vi "DIO-DAQ-Panel.vi"(7 "Set(F)":bool, 8 "error in (no error)":errorcluster, 10 "First Time(F)":bool, 11 "object in":refnum<class>) -> (0 "error out":errorcluster, 2 "Changed?":bool, 3 "object out":refnum<class>)   [LabVIEW 2021, in "DAQmx.lvlib" / "DIO-Configuration.lvclass"]
uses:
  DIO-Configuration.lvclass
  Dependencies/DIO-Channel.lvlibp/Channels/DIO-Channel/DIO-Configuration_class/tdef/Direction.ctl
  C:/Users/averna/Documents/LV Gym DEMO/Factory Pattern/Device Channels/Dependencies/DIO-Channel.lvlibp/Channels/DIO-Channel/DIO-Configuration_class/DIO-Configuration.lvclass
  tdef/Data.ctl
  DAQmx.lvlib
  Dependencies/DIO-Channel.lvlibp/Channels/DIO-Channel/DIO-Configuration_class/DIO-Configuration.lvclass
panel:
  in  "Direction":T1
  in  "Line":string(combo)
  in  "Device":string(combo)
  out "Not Saved?":bool
  in  "Save":bool
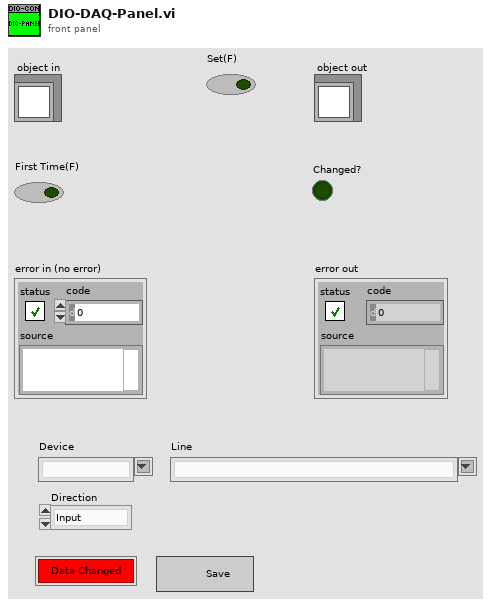
[diagram p1: front panel]
types:
  T1 = typedef "DIO-Channel.lvlibp/DIO-Configuration.lvclass/Direction.ctl" = enum16{"Input", "Output"}
  T2 = typedef "DAQmx.lvlib/DIO-Configuration.lvclass/Data.ctl" = cluster{"DAQ_Line":string}
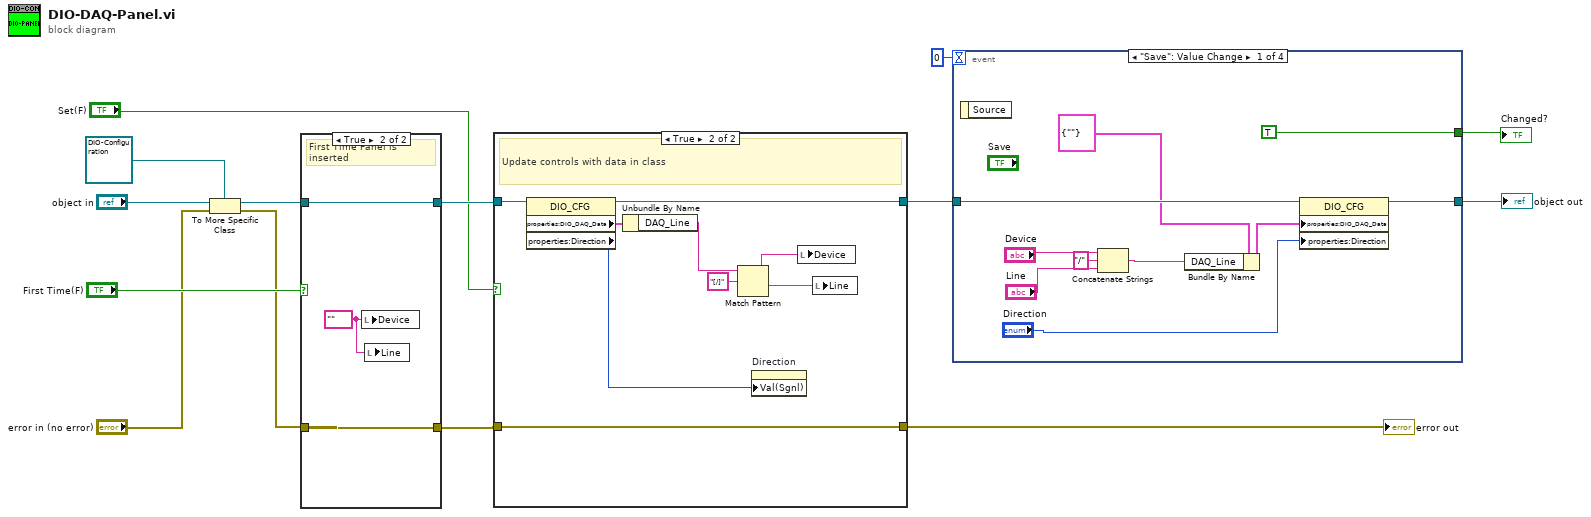
[diagram p0: block diagram]
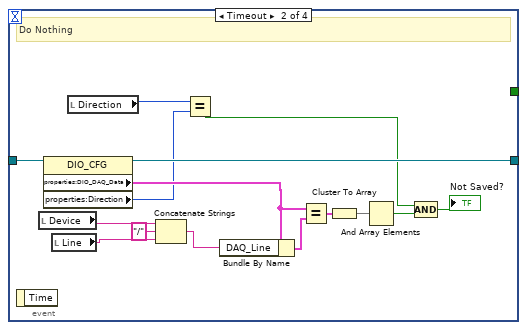
[diagram p3: hidden frame]
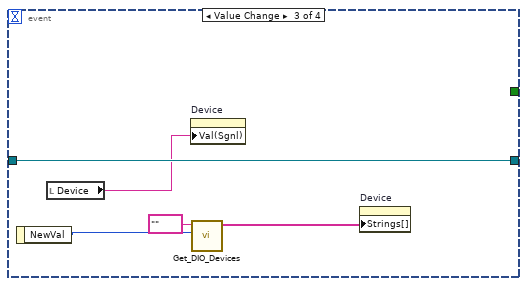
[diagram p4: hidden frame]
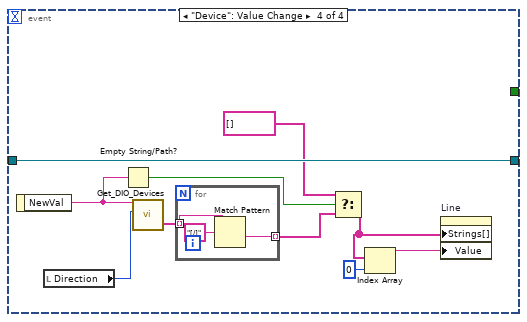
[diagram p5: hidden frame]
diagram:
  n1 = To More Specific Class(target class=refnum<class "DIO-Configuration.lvclass"> refnum ("Template-Channels.lvlib:Template_CFG"), reference="object in", error in="error in (no error)") -> (specific class reference=w8:refnum<class "DIO-Configuration.lvclass">, error out=w6:errorcluster)
  n2 = case shown="True" "First Time(F)" {
    tunnel: [w16 w19] -> w12
    tunnel: w8 -> [w16 w19]
    tunnel: [w15 w18] -> w11
    tunnel: w6 -> [w15 w18]
    frame False {
    }
    frame True {
      w17 = "" ("Device")
      # "First Time Panel is inserted"
      n3 = local write "Device"(w17) -> ()
      n4 = local write "Line"(w17) -> ()
    }
  }
  n5 = case shown="True" "Set(F)" {
    tunnel: [w21 w28] -> w3
    tunnel: w12 -> [w21 w30]
    tunnel: [w20 w29] -> w10
    tunnel: w11 -> [w20 w29]
    frame False {
    }
    frame True {
      # "Update controls with data in class"
      n6 = property class="DIO_CFG"(reference=w30) -> (reference out=w28:refnum<class "DIO-Configuration.lvclass">, "properties:DIO_DAQ_Data"=w27:T2, "properties:Direction"=w22:T1)  [unwired: 1 in, 1 out]
      n7 = Unbundle By Name(w27) -> ("DAQ_Line"=w26:string)
      n8 = Match Pattern(string=w26, regular expression="[/]") -> (before substring=w24:string, after substring=w23:string)  [unwired: 1 in, 2 out]
      n9 = property on="Direction" class="Enum (strict)"("Val(Sgnl)"=w22) -> ()  [unwired: 2 in, 2 out]
      n10 = local write "Device"(w24) -> ()
      n11 = local write "Line"(w23) -> ()
    }
  }
  "error out" <- w10
  n12 = event shown="[0] \"Save\": Value Change" {
    selector: _ -> [_ _ _ _]
    dyn-events: _ -> [_ _ _ _]
    timeout: 0 -> [_ _ _ _]
    tunnel: [w40 w54 w60 w70] -> w4
    tunnel: w3 -> [w39 w55 w60 w70]
    tunnel: [TRUE ("Changed?") _ _ _] -> w1
    event "Save": Value Change {
      n13 = event-data() -> ()  [unwired: 1 in, 1 out]
      n14 = Concatenate Strings("Device", "/" ("string"), "Line") -> (w32:string)
      n15 = Bundle By Name(cluster=T2 {"DAQ_Line"=""} ("DIO_Data"), "DAQ_Line"=w32) -> (w33:T2)
      n16 = property class="DIO_CFG"(reference=w39, "properties:DIO_DAQ_Data"=w33, "properties:Direction"="Direction") -> (reference out=w40:refnum<class "DIO-Configuration.lvclass">)  [unwired: 1 in, 1 out]
    }
    event Timeout {
      # "Do Nothing"
      n17 = event-data() -> ()  [unwired: 1 in, 1 out]
      n18 = local read "Device"() -> (w48:string)
      n19 = property class="DIO_CFG"(reference=w55) -> (reference out=w54:refnum<class "DIO-Configuration.lvclass">, "properties:DIO_DAQ_Data"=w50:T2, "properties:Direction"=w43:T1)  [unwired: 1 in, 1 out]
      n20 = local read "Line"() -> (w47:string)
      n21 = local read "Direction"() -> (w44:T1)
      n22 = Concatenate Strings(w48, "/" ("string"), w47) -> (w45:string)
      n23 = Equal?(x=w44, y=w43) -> (x = y?=w41:bool)
      n24 = Bundle By Name(cluster=w50, "DAQ_Line"=w45) -> (w49:T2)
      n25 = Equal?(x=w50, y=w49) -> (x = y?=w53:cluster{"DAQ_Line":bool})
      n26 = Cluster To Array(cluster=w53) -> (array=w52:bool[])
      n27 = And Array Elements(Boolean array=w52) -> (logical AND=w51:bool)
      n28 = Compound Arithmetic op=AND(w41, w51) -> (→"Not Saved?":bool)
    }
    event Value Change {
      n29 = event-data() -> ("NewVal"=w59:T1)  [unwired: 1 in]
      n30 = local read "Device"() -> (w57:string)
      n31 = property on="Device" class="CmbBox"("Val(Sgnl)"=w57) -> ()  [unwired: 2 in, 2 out]
      n32 = call "Get_DIO_Devices.vi"("Direction"=w59, "Device"=tag "") -> ("Devices"=w58:tag[])  [unwired: 7 in, 2 out]
      n33 = property on="Device" class="CmbBox"("Strings[]"=w58) -> ()  [unwired: 2 in, 2 out]
    }
    event "Device": Value Change {
      n34 = event-data() -> ("NewVal"=w65:string)  [unwired: 1 in]
      n35 = local read "Direction"() -> (w66:T1)
      n36 = Empty String/Path?(string/path=w65) -> (empty?=w62:bool)
      n37 = call "Get_DIO_Devices.vi"("Direction"=w66, "Device"=w65) -> ("Lines"=w67:tag[])  [unwired: 7 in, 2 out]
      n38 = for {
        tunnel: [w72] -> w63 mode=indexing
        tunnel: w67 -> [w71] mode=indexing
        n39 = Match Pattern(string=w71, regular expression="[/]") -> (after substring=w72:string)  [unwired: 1 in, 3 out]
      }
      n40 = Select(t=string[] [], s=w62, f=w63) -> (s? t:f=w64:string[])
      n41 = Index Array(array=w64, index=0) -> (element=w69:string)
      n42 = property on="Line" class="CmbBox"("Strings[]"=w64, "Value"=w69) -> ()  [unwired: 2 in, 2 out]
    }
  }
  "object out" <- w4
  "Changed?" <- w1
